vi "UI Updater Global.vi"() -> ()   [LabVIEW 2018, in "GLog.lvlib" / "UI Updater.lvlib"]
uses:
  UI Updater.lvlib
panel:
  in  "UI Updater VI Ref":refnum<vi>
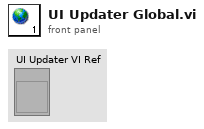
[diagram p1: front panel]
diagram:
